vi "Diff_Drive_System_Dash_Write.vi"   [LabVIEW 2019]
uses:
  Diff_Drive_System_Globals.vi
  <vilib>/Rock Robotics/Network Tables/NT Write Numeric Array.vi
  <vilib>/Rock Robotics/Network Tables/NT Write Number.vi
  <vilib>/Rock Robotics/Network Tables/NT Write Boolean.vi
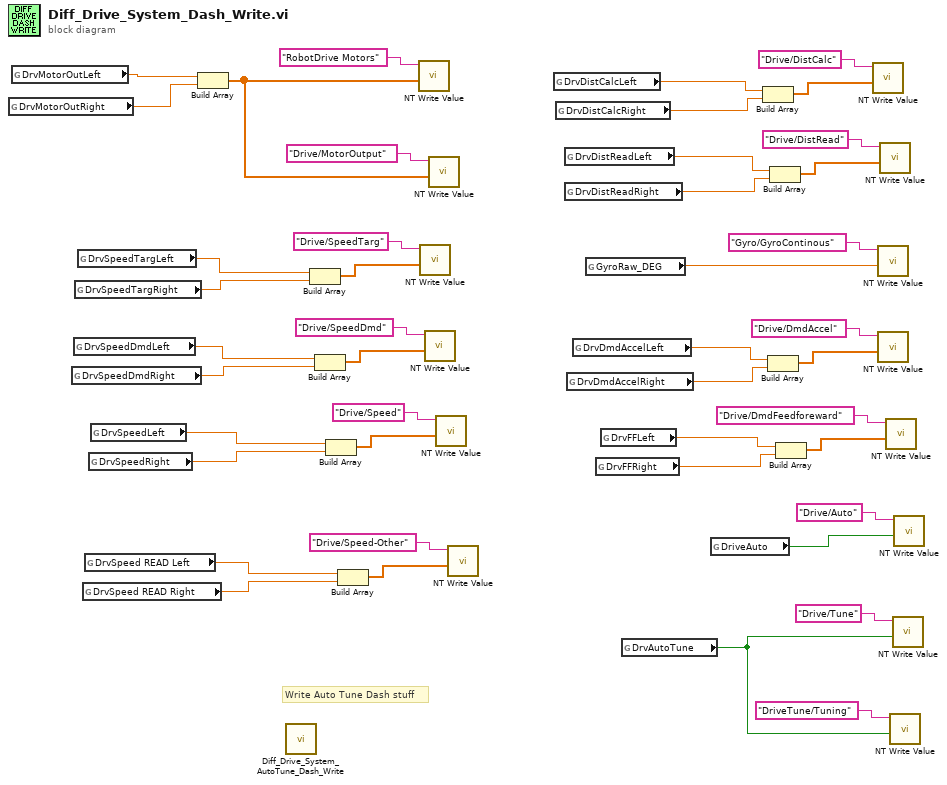
[diagram p0: block diagram]
diagram:
  # "Write Auto Tune Dash stuff"
  n1 = global read "Diff_Drive_System_Globals.vi" "DrvMotorOutRight"() -> (w26:dbl)
  n2 = global read "Diff_Drive_System_Globals.vi" "DrvMotorOutLeft"() -> (w27:dbl)
  n3 = global read "Diff_Drive_System_Globals.vi" "DrvSpeedDmdRight"() -> (w21:dbl)
  n4 = global read "Diff_Drive_System_Globals.vi" "DrvSpeedDmdLeft"() -> (w22:dbl)
  n5 = global read "Diff_Drive_System_Globals.vi" "DrvSpeedTargRight"() -> (w23:dbl)
  n6 = global read "Diff_Drive_System_Globals.vi" "DrvSpeedTargLeft"() -> (w24:dbl)
  n7 = global read "Diff_Drive_System_Globals.vi" "DrvSpeed READ Right"() -> (w6:dbl)
  n8 = global read "Diff_Drive_System_Globals.vi" "DrvSpeed READ Left"() -> (w7:dbl)
  n9 = global read "Diff_Drive_System_Globals.vi" "DrvSpeedRight"() -> (w19:dbl)
  n10 = global read "Diff_Drive_System_Globals.vi" "DrvSpeedLeft"() -> (w20:dbl)
  n11 = Build Array(w27, w26) -> (w25:dbl[])
  n12 = call "Diff_Drive_System_AutoTune_Dash_Write.vi"() -> ()  [unwired: 12 in]
  n13 = Build Array(w24, w23) -> (w30:dbl[])
  n14 = Build Array(w22, w21) -> (w32:dbl[])
  n15 = Build Array(w20, w19) -> (w34:dbl[])
  n16 = Build Array(w7, w6) -> (w8:dbl[])
  n17 = call-poly <vilib>:"NT Write Value.vi"("Numeric Array"=w25, "Name"="RobotDrive Motors") -> ()  [unwired: 9 in, 1 out]
  n18 = call-poly <vilib>:"NT Write Value.vi"("Numeric Array"=w30, "Name"="Drive/SpeedTarg") -> ()  [unwired: 9 in, 1 out]
  n19 = call-poly <vilib>:"NT Write Value.vi"("Numeric Array"=w32, "Name"="Drive/SpeedDmd") -> ()  [unwired: 9 in, 1 out]
  n20 = call-poly <vilib>:"NT Write Value.vi"("Numeric Array"=w25, "Name"="Drive/MotorOutput") -> ()  [unwired: 9 in, 1 out]
  n21 = call-poly <vilib>:"NT Write Value.vi"("Numeric Array"=w34, "Name"="Drive/Speed") -> ()  [unwired: 9 in, 1 out]
  n22 = call-poly <vilib>:"NT Write Value.vi"("Numeric Array"=w8, "Name"="Drive/Speed-Other") -> ()  [unwired: 9 in, 1 out]
  n23 = global read "Diff_Drive_System_Globals.vi" "DrvDistCalcLeft"() -> (w18:dbl)
  n24 = global read "Diff_Drive_System_Globals.vi" "DrvDistCalcRight"() -> (w17:dbl)
  n25 = global read "Diff_Drive_System_Globals.vi" "DrvDistReadLeft"() -> (w16:dbl)
  n26 = global read "Diff_Drive_System_Globals.vi" "DrvDistReadRight"() -> (w15:dbl)
  n27 = global read "Diff_Drive_System_Globals.vi" "DrvDmdAccelRight"() -> (w12:dbl)
  n28 = global read "Diff_Drive_System_Globals.vi" "DrvDmdAccelLeft"() -> (w13:dbl)
  n29 = global read "Diff_Drive_System_Globals.vi" "GyroRaw_DEG"() -> (w14:dbl)
  n30 = global read "Diff_Drive_System_Globals.vi" "DrvFFRight"() -> (w10:dbl)
  n31 = global read "Diff_Drive_System_Globals.vi" "DrvFFLeft"() -> (w11:dbl)
  n32 = global read "Diff_Drive_System_Globals.vi" "DrvAutoTune"() -> (w1:bool)
  n33 = global read "Diff_Drive_System_Globals.vi" "DriveAuto"() -> (w4:bool)
  n34 = Build Array(w18, w17) -> (w36:dbl[])
  n35 = Build Array(w13, w12) -> (w41:dbl[])
  n36 = Build Array(w16, w15) -> (w38:dbl[])
  n37 = Build Array(w11, w10) -> (w43:dbl[])
  n38 = call-poly <vilib>:"NT Write Value.vi"("Numeric Array"=w36, "Name"="Drive/DistCalc") -> ()  [unwired: 9 in, 1 out]
  n39 = call-poly <vilib>:"NT Write Value.vi"("Numeric"=w14, "Name"="Gyro/GyroContinous") -> ()  [unwired: 9 in, 1 out]
  n40 = call-poly <vilib>:"NT Write Value.vi"("Numeric Array"=w41, "Name"="Drive/DmdAccel") -> ()  [unwired: 9 in, 1 out]
  n41 = call-poly <vilib>:"NT Write Value.vi"("Numeric Array"=w38, "Name"="Drive/DistRead") -> ()  [unwired: 9 in, 1 out]
  n42 = call-poly <vilib>:"NT Write Value.vi"("Numeric Array"=w43, "Name"="Drive/DmdFeedforeward") -> ()  [unwired: 9 in, 1 out]
  n43 = call-poly <vilib>:"NT Write Value.vi"("Boolean"=w1, "Name"="DriveTune/Tuning") -> ()  [unwired: 9 in, 1 out]
  n44 = call-poly <vilib>:"NT Write Value.vi"("Boolean"=w1, "Name"="Drive/Tune") -> ()  [unwired: 9 in, 1 out]
  n45 = call-poly <vilib>:"NT Write Value.vi"("Boolean"=w4, "Name"="Drive/Auto") -> ()  [unwired: 9 in, 1 out]
